vi "D4xxx Get STB - beta.vi"() -> ()   [LabVIEW 2009]
panel:
  out "Error message":string
  in  "error in (no error)":errorcluster
  out "error out":errorcluster
  in  "VISA resource name":refnum<visa-resource-name>
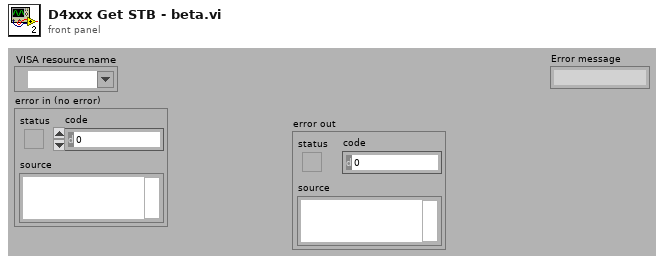
[diagram p1: front panel]
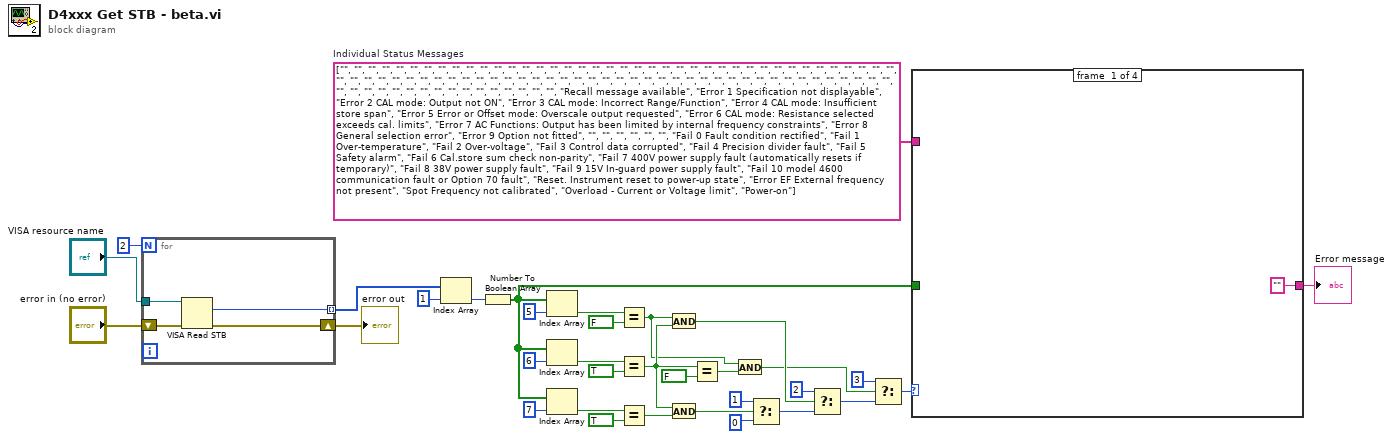
[diagram p0: block diagram]
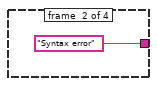
[diagram p2: hidden frame]
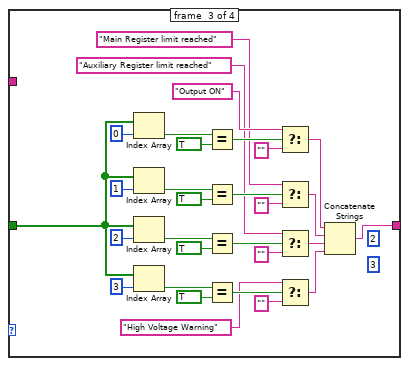
[diagram p3: hidden frame]
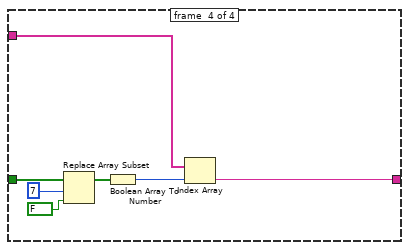
[diagram p4: hidden frame]
diagram:
  w1 = string[] ["", "", "", "", "", "", "", "", "", "", "", "", "", "", "", "", "", "", "", "", "", "", "", "", "", "", "", "", "", "", "", "", "", "", "", "", "", "", "", "", "", "", "", "", "", "", "", "", "", "", "", "", "", "", "", "", "", "", "", "", "", "", "", "", "", "", "", "", "", "", "", "", "", "", "", "", "", "", "", "", "", "", "", "", "", "", "", "", "", "", "", "", "", "", "", "", "Recall message available", "Error 1 Specification not displayable", "Error 2 CAL mode: Output not ON", "Error 3 CAL mode: Incorrect Range/Function", "Error 4 CAL mode: Insufficient store span", "Error 5 Error or Offset mode: Overscale output requested", "Error 6 CAL mode: Resistance selected exceeds cal. limits", "Error 7 AC Functions: Output has been limited by internal frequency constraints", "Error 8 General selection error", "Error 9 Option not fitted", "", "", "", "", "", "", "Fail 0 Fault condition rectified", "Fail 1 Over-temperature", "Fail 2 Over-voltage", "Fail 3 Control data corrupted", "Fail 4 Precision divider fault", "Fail 5 Safety alarm", "Fail 6 Cal.store sum check non-parity", "Fail 7 400V power supply fault (automatically resets if temporary)", "Fail 8 38V power supply fault", "Fail 9 15V In-guard power supply fault", "Fail 10 model 4600 communication fault or Option 70 fault", "Reset. Instrument reset to power-up state", "Error EF External frequency not present", "Spot Frequency not calibrated", "Overload - Current or Voltage limit", "Power-on"]  # Individual Status Messages
  n1 = for {
    N: 2 -> [_]
    tunnel: "VISA resource name" -> [w38]
    shift-right: [w37] -> w33
    shift-left: "error in (no error)" -> [w36]
    tunnel: [w35] -> w30 mode=indexing
    n2 = VISA Read STB(8:w36, 11:w38) -> (0:w37:errorcluster, 2:w35:u16)  [unwired: 1 out]
  }
  "error out" <- w33
  n3 = Index Array(array=w30, index=1) -> (element=w28:u16)
  n4 = Number To Boolean Array(number=w28) -> (Boolean array=w3:bool[])
  n5 = Index Array(array=w3, index=5) -> (element=w17:bool)
  n6 = Index Array(array=w3, index=6) -> (element=w25:bool)
  n7 = Index Array(array=w3, index=7) -> (element=w23:bool)
  n8 = Equal?(x=w17, y=FALSE) -> (x = y?=w8:bool)
  n9 = Equal?(x=w25, y=TRUE) -> (x = y?=w10:bool)
  n10 = Equal?(x=w23, y=TRUE) -> (x = y?=w21:bool)
  n11 = And(x=w8, y=w10) -> (x .and. y?=w12:bool)
  n12 = And(x=w10, y=w21) -> (x .and. y?=w20:bool)
  n13 = Equal?(x=w10, y=FALSE) -> (x = y?=w9:bool)
  n14 = And(x=w8, y=w9) -> (x .and. y?=w5:bool)
  n15 = Select(t=1, s=w20, f=0) -> (s? t:f=w13:i32)
  n16 = Select(t=2, s=w12, f=w13) -> (s? t:f=w6:i32)
  n17 = Select(t=3, s=w5, f=w6) -> (s? t:f=w4:i32)
  n18 = case shown="2" w4 {
    tunnel: w3 -> [_ _ w56 w74]
    tunnel: w1 -> [_ _ _ w73]
    tunnel: ["" "Syntax error" w43 w71] -> w2
    frame #0 {
    }
    frame #1 {
    }
    frame #2 {
      (unwired) 3 ("index")
      (unwired) 2 ("index")
      n19 = Index Array(array=w56, index=0) -> (element=w69:bool)
      n20 = Index Array(array=w56, index=1) -> (element=w65:bool)
      n21 = Index Array(array=w56, index=2) -> (element=w55:bool)
      n22 = Index Array(array=w56, index=3) -> (element=w54:bool)
      n23 = Equal?(x=w69, y=TRUE) -> (x = y?=w67:bool)
      n24 = Equal?(x=w65, y=TRUE) -> (x = y?=w63:bool)
      n25 = Equal?(x=w55, y=TRUE) -> (x = y?=w53:bool)
      n26 = Equal?(x=w54, y=TRUE) -> (x = y?=w52:bool)
      n27 = Select(t="Output ON", s=w67, f="") -> (s? t:f=w60:string)
      n28 = Select(t="Main Register limit reached", s=w63, f="") -> (s? t:f=w57:string)
      n29 = Select(t="Auxiliary Register limit reached", s=w53, f="") -> (s? t:f=w45:string)
      n30 = Select(t="High Voltage Warning", s=w52, f="") -> (s? t:f=w44:string)
      n31 = Concatenate Strings(w60, w57, w45, w44) -> (w43:string)
    }
    frame #3 {
      n32 = Replace Array Subset(array=w74, new element=FALSE ("new element/subarray"), index=7) -> (w75:bool[])
      n33 = Boolean Array To Number(Boolean array=w75) -> (number=w72:u32)
      n34 = Index Array(array=w73, index=w72) -> (element=w71:string)
    }
  }
  "Error message" <- w2
